vi "DVR Insert Control By Reference.vi"(8 "error in (no error)":errorcluster, 11 "Ctl Refnum":refnum<vi>) -> (0 "error out":errorcluster)   [LabVIEW 2019, in "Language Selection.lvlib"]
doc: "- - -\nCopyright (c) 2026, Merecs Engineering GmbH"
uses:
  Language Selection.lvlib
  <vilib>/Utility/miscctls.llb/LVMapReplaceAction.ctl
  Global Language Selection.vi
panel:
  # "Connector Pane"
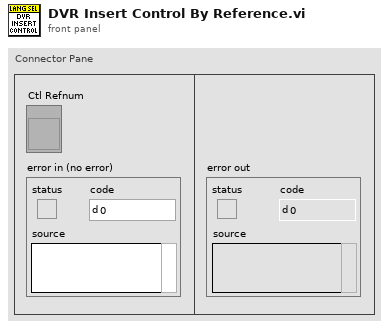
[diagram p1: front panel]
types:
  T1 = typedef "LVMapReplaceAction.ctl" = enum32{"Modify Entry only if found", "Add or Modify Entry", "Delete Entry"}
  T2 = typedef "Language Selection.lvlib/Cluster DVR.ctl" = cluster{"Data":T3, "VIs":path[], "FP Translation":map{string, T4}, "Text Translation":map{string, T4}, "Front panels":set{refnum<vi>}}
  T3 = typedef "Language Selection.lvlib/Cluster Settings Data.ctl" = cluster{"Startup Language":string, "Default Language":string, "Languages":cluster{"ANSI":string[], "Unicode":string[]}}
  T4 = typedef "Language Selection.lvlib/Cluster LanguageClusterWithRefnum.ctl" = cluster{"Property":T5[], "Controls":set{refnum<vi>}}
  T5 = typedef "Language Selection.lvlib/Cluster PropertyTranslation.ctl" = cluster{"Type":T6, "Translation ANSI":string[], "Translation Unicode":string[]}
  T6 = typedef "Language Selection.lvlib/Enum Property Type.ctl" = enum16{"NA", "Caption", "String Value", "Boolean Text", "Ring Strings", "1D Array Elements", "2D Array Elements", "(MC)Listbox Header", "(MC)Listbox Items", "Tab Pages Names", "X & Y GraphChart", "Plot Names", "Table Headers", "Table Items", "TipStrip", "Combobox Strings", "Cursor Name", "Tree Col Headers"}
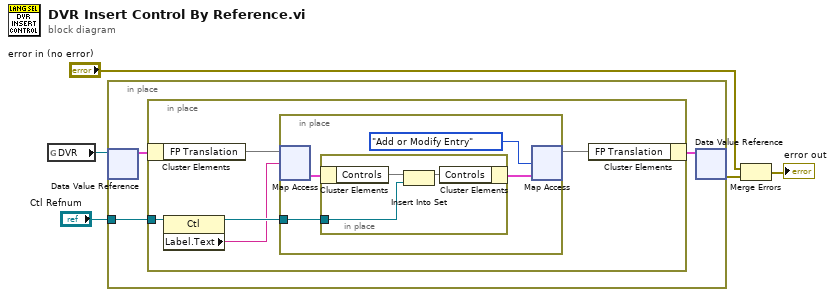
[diagram p0: block diagram]
diagram:
  n1 = global read "Global Language Selection.vi" "DVR"() -> (w4:refnum<data-value>)
  n2 = in-place {
    in-place-border: "Ctl Refnum" -> [w8]
    n3 = in-place-dvr #1(w4) -> (w7:T2)  [unwired: 1 out]
    n4 = in-place {
      in-place-border: w8 -> [w13]
      n5 = in-place-cluster #2(w7) -> ("FP Translation"=w11:map{string, T4})
      n6 = property class="Ctl"(reference=w13) -> (reference out=w12:refnum<vi>, "Label.Text"=w10:string)  [unwired: 1 in, 1 out]
      n7 = in-place {
        in-place-border: w12 -> [w17]
        n8 = in-place-map #3(w11, w10) -> (w15:T4)  [unwired: 1 in, 1 out]
        n9 = in-place {
          in-place-border: w17 -> [w18]
          n10 = in-place-cluster #4(w15) -> ("Controls"=w20:set{refnum<vi>})
          n11 = Insert Into Set(10:w18, 11:w20) -> (3:w19:set{refnum<vi>})  [unwired: 1 out]
          n12 = in-place-cluster #4("Controls"=w19) -> (w14:T4)
        }
        n13 = in-place-map #3(w14, LVMapReplaceAction."Add or Modify Entry" ("action")) -> (w9:map{string, T4})  [unwired: 2 out]
      }
      n14 = in-place-cluster #2("FP Translation"=w9) -> (w6:T2)
    }
    n15 = in-place-dvr #1(w6) -> (w2:errorcluster)  [unwired: 1 out]
  }
  n16 = Merge Errors("error in (no error)", w2) -> (→"error out":errorcluster)
